vi "Write Batch OD By Array Index - i16.vi"(8 "error in (no error)":errorcluster, 9 "value":i16, 10 "array index":i32, 11 "OD Batch in":refnum<class "OD Batch.lvclass">) -> (0 "error out":errorcluster, 3 "OD Batch out":refnum<class "OD Batch.lvclass">)   [LabVIEW 2023, in "xnet_canopen.lvlib" / "OD Batch.lvclass"]
uses:
  OD Batch.lvclass
  OD Batch.lvclass/OD Batch.ctl
  typedef/canopen types.ctl
  xnet_canopen.lvlib
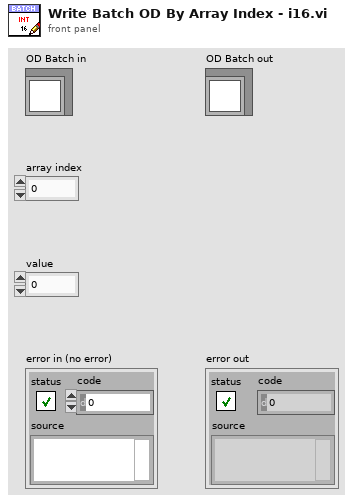
[diagram p1: front panel]
types:
  T1 = typedef "xnet_canopen.lvlib/od entry.ctl" = cluster{"OD Index":T2, "CANOpen Types":T3, "Size":u32, "Offset":u32, "Value":variant, "Initialized":bool}
  T2 = typedef "xnet_canopen.lvlib/od index.ctl" = cluster{"Index":u16, "SubIndex":u8}
  T3 = typedef "xnet_canopen.lvlib/canopen types.ctl" = u32
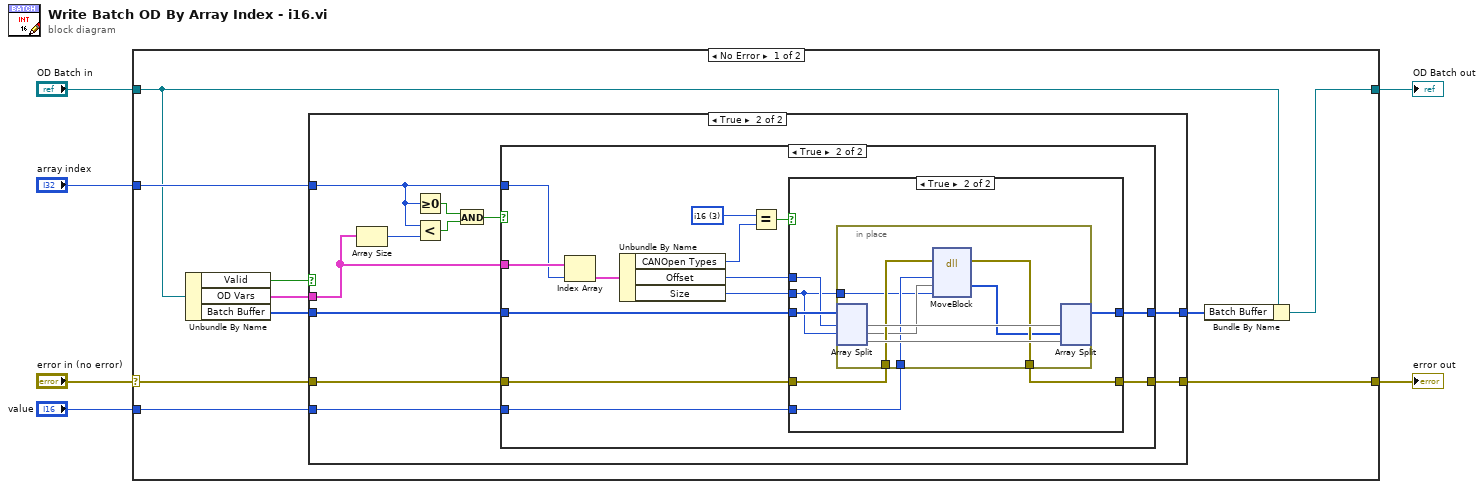
[diagram p0: block diagram]
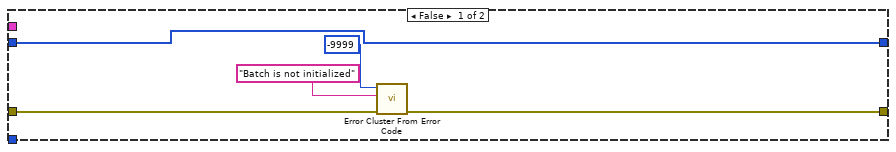
[diagram p2: hidden frame]
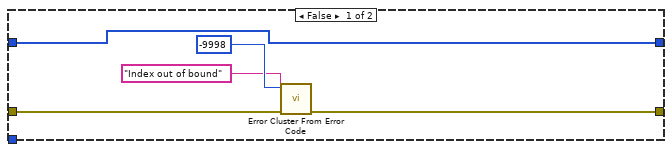
[diagram p3: hidden frame]
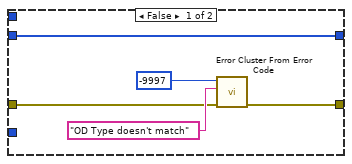
[diagram p4: hidden frame]
diagram:
  n1 = case shown="No Error" "error in (no error)" {
    selector: "error in (no error)" -> [w16 w72]
    tunnel: [w15 w72] -> w5
    tunnel: [w8 w71] -> w3
    tunnel: "OD Batch in" -> [w9 w71]
    tunnel: "array index" -> [w12 _]
    tunnel: "value" -> [w10 _]
    frame No Error {
      n2 = Unbundle By Name(w9) -> ("Valid"=w14:bool, "OD Vars"=w13:T1[], "Batch Buffer"=w11:u8[])
      n3 = case shown="True" w14 {
        tunnel: w16 -> [w21 w26]
        tunnel: [w20 w25] -> w15
        tunnel: w13 -> [_ w32]
        tunnel: w12 -> [_ w30]
        tunnel: w11 -> [w17 w24]
        tunnel: w10 -> [_ w23]
        tunnel: [w17 w22] -> w7
        frame False {
          n4 = call <vilib>:"Error Cluster From Error Code.vi"("error in (no error)"=w21, "error message (\"\")"="Batch is not initialized" ("error message (\"\")"), "error code (0)"=-9999) -> ("error out"=w20:errorcluster)  [unwired: 6 in]
        }
        frame True {
          n5 = Array Size(array=w32) -> (size(s)=w31:i32)
          n6 = Greater Or Equal To 0?(x=w30) -> (x >= 0?=w28:bool)
          n7 = Less?(x=w30, y=w31) -> (x < y?=w29:bool)
          n8 = And(x=w28, y=w29) -> (x .and. y?=w27:bool)
          n9 = case shown="True" w27 {
            tunnel: w32 -> [_ w50]
            tunnel: w30 -> [_ w49]
            tunnel: w26 -> [w35 w46]
            tunnel: [w34 w45] -> w25
            tunnel: w24 -> [w33 w44]
            tunnel: w23 -> [_ w39]
            tunnel: [w33 w38] -> w22
            frame False {
              n10 = call <vilib>:"Error Cluster From Error Code.vi"("error in (no error)"=w35, "error message (\"\")"="Index out of bound" ("error message (\"\")"), "error code (0)"=-9998) -> ("error out"=w34:errorcluster)  [unwired: 6 in]
            }
            frame True {
              w40 = T3 3 items=["bool"=1, "i8"=2, "i16"=3, "i32"=4, "u8"=5, "u16"=6, "u32"=7, "f32"=8, "visible str"=9, "octet str"=10, "f64"=17, "i64"=21, "u64"=27] ("CANOpen Types")
              n11 = Index Array(array=w50, index=w49) -> (element=w48:T1)
              n12 = Unbundle By Name(w48) -> ("CANOpen Types"=w41:T3, "Offset"=w43:u32, "Size"=w42:u32)
              n13 = Equal?(x=w40, y=w41) -> (x = y?=w47:bool)
              n14 = case shown="True" w47 {
                tunnel: w46 -> [w53 w60]
                tunnel: [w52 w59] -> w45
                tunnel: w44 -> [w51 w62]
                tunnel: w43 -> [_ w61]
                tunnel: w42 -> [_ w57]
                tunnel: w39 -> [_ w58]
                tunnel: [w51 w56] -> w38
                frame False {
                  n15 = call <vilib>:"Error Cluster From Error Code.vi"("error in (no error)"=w53, "error message (\"\")"="OD Type doesn't match" ("error message (\"\")"), "error code (0)"=-9997) -> ("error out"=w52:errorcluster)  [unwired: 6 in]
                }
                frame True {
                  n16 = in-place {
                    in-place-border: w60 -> [w68]
                    in-place-border: [w67] -> w59
                    in-place-border: w58 -> [w65]
                    in-place-border: w57 -> [w64]
                    n17 = in-place-split #1(w62, w61, w57) -> (w70:u8[], w66:u8[], w69:u8[])
                    n18 = dll-call lib="LabVIEW" fn="MoveBlock"(error in=w68, "src"=w65, "dst"=w66, "sz"=w64) -> (error out=w67:errorcluster, "dst"=w63:u8[])  [unwired: 5 in, 1 out]
                    n19 = in-place-split #1(w70, w63, w69) -> (w56:u8[])  [unwired: 2 out]
                  }
                }
              }
            }
          }
        }
      }
      n20 = Bundle By Name(cluster=w9, "Batch Buffer"=w7) -> (w8:refnum<class "OD Batch.lvclass">)
    }
    frame Error {
    }
  }
  "error out" <- w5
  "OD Batch out" <- w3
